vi "set Trace Mode.vi"(8 "error in (no error)":errorcluster, 9 "Trace Index":u32=1 min=1, 10 "Trace Mode":T1, 11 "Keysight 9020A in":refnum<class "Keysight 9020A.lvclass">) -> (0 "error out":errorcluster, 3 "Keysight 9020A out":refnum<class "Keysight 9020A.lvclass">)   [LabVIEW 2023, in "Spectrum Analyzer.lvlib" / "Keysight 9020A.lvclass"]
uses:
  Keysight 9020A.lvclass
  TYPE DEFINITION/TYPE Display Trace Mode Select.ctl
  Keysight 9020A.lvclass/Keysight 9020A.ctl
  Spectrum Analyzer.lvlib
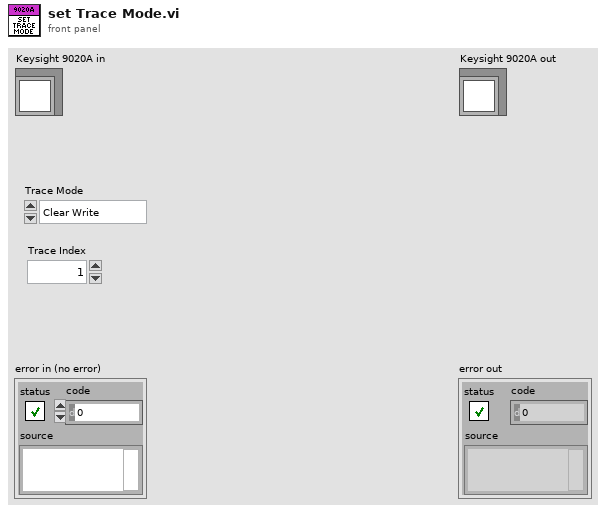
[diagram p1: front panel]
types:
  T1 = typedef "Spectrum Analyzer.lvlib/TYPE Display Trace Mode Select.ctl" = enum16{"Clear Write", "Max Hold", "Min Hold", "Average", "View"}
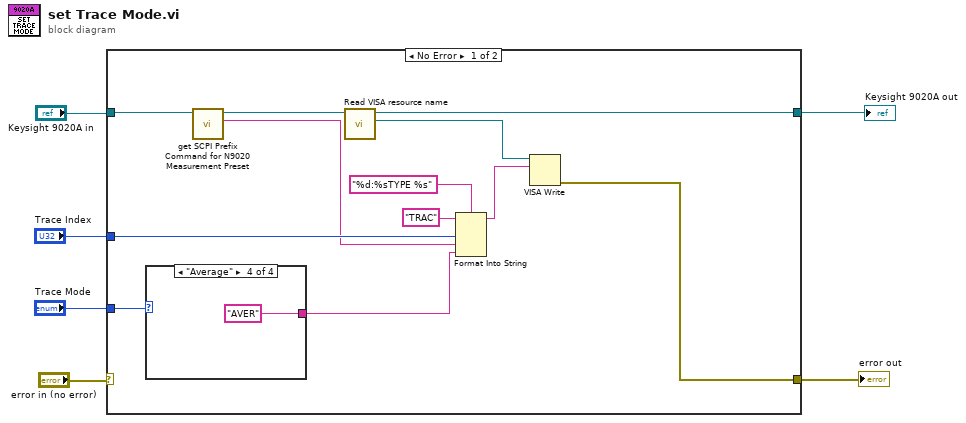
[diagram p0: block diagram]
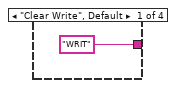
[diagram p2: hidden frame]
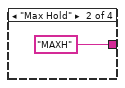
[diagram p3: hidden frame]
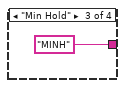
[diagram p4: hidden frame]
diagram:
  n1 = case shown="No Error" "error in (no error)" {
    selector: "error in (no error)" -> [_ w23]
    tunnel: "Keysight 9020A in" -> [w11 w24]
    tunnel: [w18 w24] -> w5
    tunnel: [w15 w23] -> w3
    tunnel: "Trace Mode" -> [w14 _]
    tunnel: "Trace Index" -> [w13 _]
    frame No Error {
      n2 = case shown="\"Average\"" w14 {
        tunnel: ["WRIT" "MAXH" "MINH" "AVER"] -> w8
        frame "Clear Write", Default {
        }
        frame "Max Hold" {
        }
        frame "Min Hold" {
        }
        frame "Average" {
        }
      }
      n3 = call "get SCPI Prefix Command for N9020 Measurement Preset.vi"("Keysight 9020A in"=w11) -> ("SCPI Prefix Command"=w7:string, "Keysight 9020A out"=w10:refnum<class "Keysight 9020A.lvclass">)  [unwired: 8 in, 1 out]
      n4 = call "Read VISA resource name.vi"("Keysight 9020A in"=w10) -> ("VISA resource name"=w16:refnum<visa-resource-name>, "Keysight 9020A out"=w18:refnum<class "Keysight 9020A.lvclass">)  [unwired: 8 in, 1 out]
      n5 = Format Into String(format string="%d:%sTYPE %s", initial string="TRAC", w13, w7, w8) -> (resulting string=w12:string)  [unwired: 1 in, 1 out]
      n6 = VISA Write(VISA resource name=w16, write buffer=w12) -> (error out=w15:errorcluster)  [unwired: 1 in, 2 out]
    }
    frame Error {
    }
  }
  "error out" <- w3
  "Keysight 9020A out" <- w5
